vi "Mouse Monitor.vi"(10 "Mouse Up (Outside Pane)":refnum<user-event>, 11 "Initial State":bool[](array[boolean])) -> ()   [LabVIEW 2019]
uses:
  <vilib>/Utility/inputDevices.llb/mouseAcquire.vi
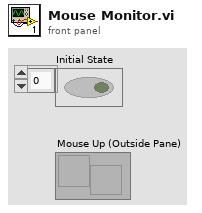
[diagram p1: front panel]
types:
  T1 = cluster{"button 1":bool, "button 2":bool, "button 3":bool, "button 4":bool}
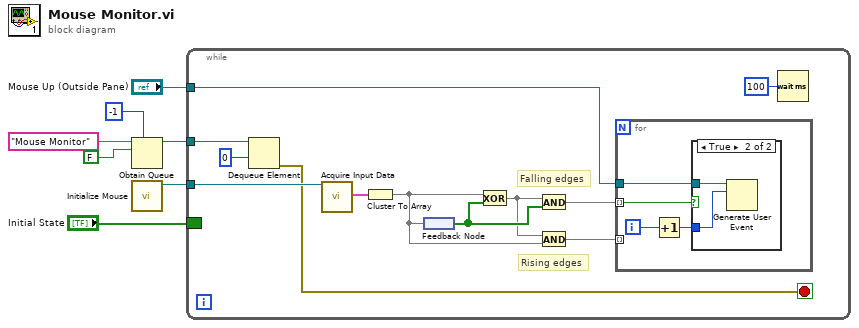
[diagram p0: block diagram]
diagram:
  n1 = Obtain Queue(max queue size (-1, unlimited)=-1, name (unnamed)="Mouse Monitor", element data type=FALSE ("create if not found? (T)")) -> (queue out=w4:refnum<queue>)  [unwired: 2 in, 2 out]
  n2 = call <vilib>:"Initialize Mouse.vi"() -> ("device ID"=w7:refnum<k1>)  [unwired: 10 in, 1 out]
  n3 = while {
    tunnel: w7 -> [w19]
    tunnel: w4 -> [w13]
    border: "Initial State" -> [_]
    tunnel: "Mouse Up (Outside Pane)" -> [w9]
    stop <- w10 stop-if-true
    # "Rising edges"
    # "Falling edges"
    n4 = Dequeue Element(queue=w13, timeout in ms (-1)=0) -> (error out=w10:errorcluster)  [unwired: 1 in, 3 out]
    n5 = call-poly <vilib>:"Acquire Input Data.vi"("device ID"=w19) -> ("button info"=w18:T1)  [unwired: 15 in, 3 out]
    n6 = Cluster To Array(cluster=w18) -> (array=w11:bool[])
    n7 = feedback #1() -> (w17:bool[])
    n8 = feedback-in #1(w11) -> ()
    n9 = Exclusive Or(1:w17, 2:w11) -> (0:w16:bool[])
    n10 = And(x=w16, y=w17) -> (x .and. y?=w15:bool[])
    n11 = And(x=w16, y=w11) -> (x .and. y?=w8:bool[])
    n12 = for {
      tunnel: w15 -> [w23] mode=indexing
      tunnel: w9 -> [w22]
      tunnel: w8 -> [_] mode=indexing
      i -> [w21]
      n13 = Increment(x=w21) -> (x+1=w20:i32)
      n14 = case shown="True" w23 {
        tunnel: w22 -> [_ w25]
        tunnel: w20 -> [_ w24]
        frame False {
        }
        frame True {
          n15 = Generate User Event(user event=w25, event data cluster=w24) -> ()  [unwired: 2 in, 2 out]
        }
      }
    }
    n16 = Wait (ms)(milliseconds to wait=u32 100) -> ()  [unwired: 1 out]
  }
